vi "Replay Loop Business Logic.vi"(11 "Replay Helper Loop In":T1) -> (3 "Replay Helper Loop Out":T1)   [LabVIEW 2026, in "dependencies.lvlib"]
uses:
  dependencies.lvlib
  User32.dll
  <userlib>/_OpenG.lib/comparison/comparison.llb/openg_comparison__ogtk.lvlib
  e6fa854f-775a-42ef-8fee-ae5b514428da.vi
  MouseLUTSelector.ctl
  ea25d2fe-5e75-4f74-a99b-35237287ff8a.vi
  <userlib>/_OpenG.lib/comparison/comparison.llb/U8 Changed__ogtk.vi
  Replay Helper Loop.ctl
panel:
  out "error out":errorcluster
  in  "error in (no error)":errorcluster
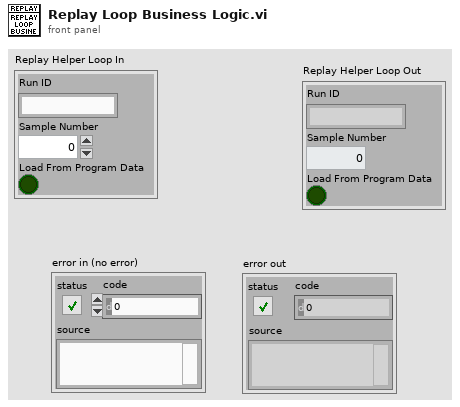
[diagram p1: front panel]
types:
  T1 = typedef "dependencies.lvlib/Replay Helper Loop.ctl" = cluster{"Run ID":string, "Sample Number":i32, "Load From Program Data":bool}
  T2 = typedef "dependencies.lvlib/MouseLUTSelector.ctl" = enum16{"Initialize", "Get Button and Axis Info", "Assign Button and Axis Info to Sample Number"}
  T3 = cluster{"Horizontal":i32, "Vertical":i32, "Scrolling":i32}
  T4 = cluster{"button 1":bool, "button 2":bool, "button 3":bool, "button 4":bool}
  T5 = typedef "dependencies.lvlib/SerializedKeyPress.ctl" = cluster{"Key Down":bool, "Key Up":bool, "Key":T6}
  T6 = typedef "dependencies.lvlib/KeyType.ctl" = enum16{"0", "1", "2", "3", "4", "5", "6", "7", "8", "9", "A", "B", "C", "D", "E", "F", "G", "H", "I", "J", "K", "L", "M", "N", "O", "P", "Q", "R", "S", "T", "U", "V", "W", "X", "Y", "Z", "F1", "F2", "F3", "F4", "F5", "F6", "F7", "F8", "F9", "F10", "F11", "F12", "F13", "F14", "F15", "ADD", "BACK", "BACKSLASH", "CAPITAL", "COMMA", "DECIMAL", "DELETE", "DIVIDE", "DOWN", "END", "EQUALS", "ESCAPE", "GRAVE (`)", "HOME", "INSERT", "LBRACKET", "LCONTROL", "LEFT", "L ALT", "LSHIFT", "LWIN", "MINUS", "MULTIPLY", "NEXT", "NUMLOCK", "NUMPAD_0", "NUMPAD_1", "NUMPAD_2", "NUMPAD_3", "NUMPAD_4", "NUMPAD_5", "NUMPAD_6", "NUMPAD_7", "NUMPAD_8", "NUMPAD_9", "PAUSE", "PERIOD", "PRIOR (PG UP)", "RBRACKET", "RCONTROL", "RETURN", "RIGHT", "R ALT", "RSHIFT", "RWIN", "SCROLL", "SEMICOLON", "SLASH", "SPACE", "SUBTRACT", "TAB", "UP", "ENTER (num pad)", "' (quote)"}
  T7 = typedef "dependencies.lvlib/KeyboardReplayKey.ctl" = u8
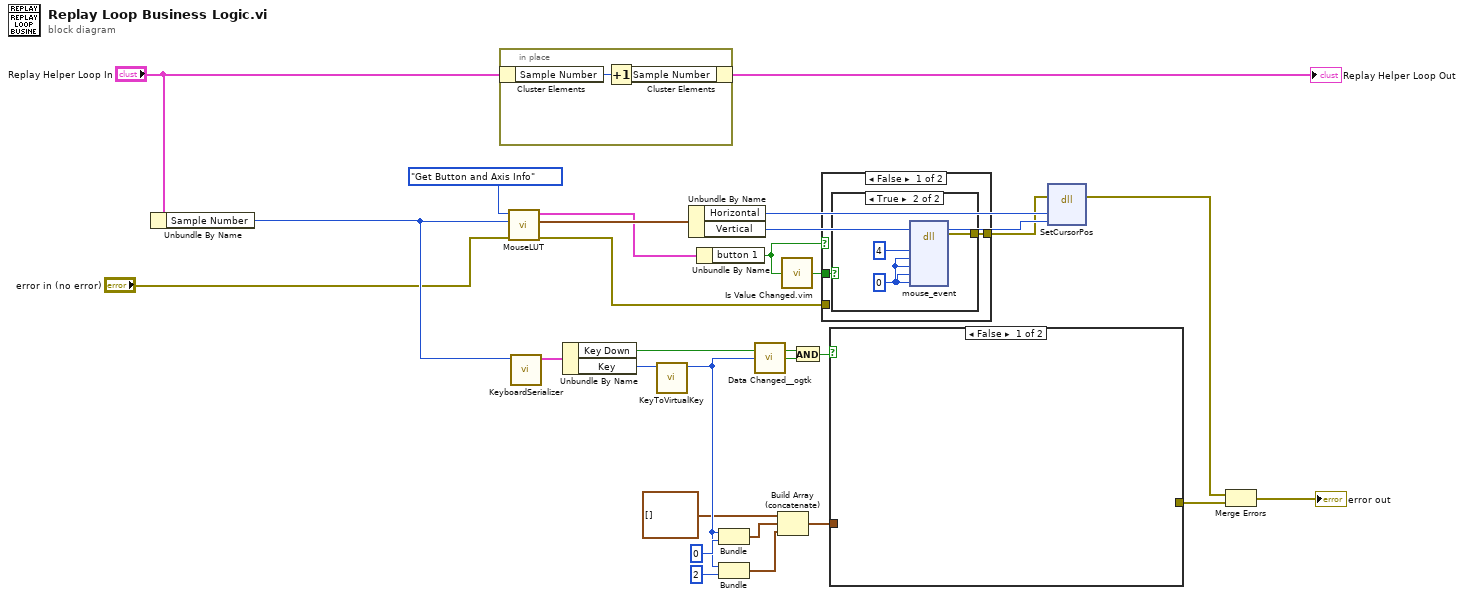
[diagram p0: block diagram]
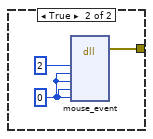
[diagram p4: hidden frame]
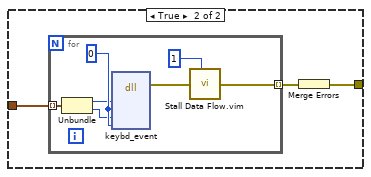
[diagram p5: hidden frame]
diagram:
  n1 = Unbundle By Name("Replay Helper Loop In") -> ("Sample Number"=w13:i32)
  n2 = in-place {
    n3 = in-place-cluster #1("Replay Helper Loop In") -> ("Sample Number"=w30:i32)
    n4 = Increment(x=w30) -> (x+1=w29:i32)
    n5 = in-place-cluster #1("Sample Number"=w29) -> (→"Replay Helper Loop Out":T1)
  }
  n6 = call "MouseLUT.vi"("error in (no error)"="error in (no error)", "Sample Number"=w13, "LUT Selector"=MouseLUTSelector."Get Button and Axis Info") -> ("error out"=w2:errorcluster, "axis info out"=w12:T3, "button info out"=w11:T4)  [unwired: 6 in]
  n7 = call "KeyboardSerializer.vi"("Sample Number"=w13) -> ("SerializedKeyPress"=w25:T5)  [unwired: 9 in, 1 out]
  n8 = Unbundle By Name(w25) -> ("Key Down"=w15:bool, "Key"=w1:T6)
  n9 = call "KeyToVirtualKey.vi"("keyType Recorded"=w1) -> ("Virtual Key"=w19:T7)  [unwired: 9 in, 1 out]
  n10 = Unbundle By Name(w12) -> ("Horizontal"=w28:i32, "Vertical"=w27:i32)
  n11 = Unbundle By Name(w11) -> ("button 1"=w26:bool)
  n12 = Bundle("Virtual Key"=w19, 0) -> (w23:cluster{"Virtual Key":T7, i32})  [unwired: 1 in]
  n13 = Bundle("Virtual Key"=w19, 2) -> (w24:cluster{"Virtual Key":T7, i32})  [unwired: 1 in]
  n14 = call-poly <userlib>:"Data Changed__ogtk.vi"("U8"=w19) -> ("Changed"=w16:bool)
  n15 = Build Array (concatenate)(cluster{i32, i32}[] [], w23, w24) -> (w20:cluster{"Virtual Key":i32, i32}[])
  n16 = call "Is Value Changed.vim"("value"=w26) -> ("changed or first call?"=w10:bool)
  n17 = And(x=w15, y=w16) -> (x .and. y?=w18:bool)
  n18 = case shown="False" w26 {
    tunnel: w10 -> [w32 w37]
    tunnel: [w31 w36] -> w8
    tunnel: w2 -> [_ _]
    frame False {
      n19 = case shown="True" w32 {
        tunnel: [_ w33] -> w31
        frame False {
        }
        frame True {
          w34 = u32 0 ("dy")
          n20 = dll-call lib="user32.dll" fn="mouse_event"("dwFlags"=u32 4, "dx"=w34, "dy"=w34, "dwData"=w34, "dwExtraInfo"=w34) -> (error out=w33:errorcluster)  [unwired: 9 in, 1 out]
        }
      }
    }
    frame True {
      n21 = case shown="False" w37 {
        tunnel: [_ w38] -> w36
        frame False {
        }
        frame True {
          w39 = u32 0 ("dy")
          n22 = dll-call lib="user32.dll" fn="mouse_event"("dwFlags"=u32 2, "dx"=w39, "dy"=w39, "dwData"=w39, "dwExtraInfo"=w39) -> (error out=w38:errorcluster)  [unwired: 9 in, 1 out]
        }
      }
    }
  }
  n23 = case shown="False" w18 {
    tunnel: w20 -> [_ w43]
    tunnel: [_ w41] -> w7
    frame False {
    }
    frame True {
      n24 = for {
        tunnel: w43 -> [w49] mode=indexing
        tunnel: [w44] -> w42 mode=indexing
        w50 = u32 0 ("dwFlags")
        n25 = Unbundle(w49) -> ("Virtual Key"=w48:i32, w47:i32)
        n26 = dll-call lib="user32.dll" fn="keybd_event"("bVk"=w48, "bScan"=w50, "dwFlags"=w47, "dwExtraInfo"=w50) -> (error out=w46:errorcluster)  [unwired: 8 in, 1 out]
        n27 = call "Stall Data Flow.vim"("value in"=w46, "milliseconds to wait"=u32 1) -> ("value out"=w44:errorcluster)  [unwired: 1 out]
      }
      n28 = Merge Errors(w42) -> (w41:errorcluster)
    }
  }
  n29 = dll-call lib="User32.dll" fn="SetCursorPos" label="SetCursorPos (User32.dll)"(error in=w8, w28, w27) -> (error out=w6:errorcluster)  [unwired: 4 in, 2 out]
  n30 = Merge Errors(w6, w7) -> (→"error out":errorcluster)
